vi "Save Image Module.vi"(8 "error in":errorcluster, 10 "Data":u64[](array[numeric]), 11 "Mode":T1) -> (0 "error out":errorcluster, 3 "File Open?":bool)   [LabVIEW 2013]
uses:
  Save Image Module Enum.ctl
  Debug/Debug Settings FG Enum.ctl
  Image Acquisition/Image Acquisition Settings FG Enum.ctl
  Image Processing/Mask ROI FG Enum.ctl
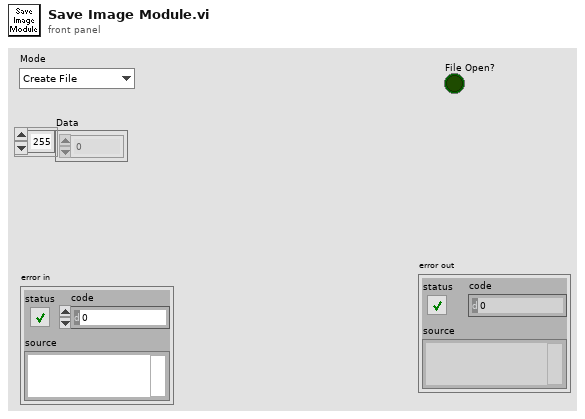
[diagram p1: front panel]
types:
  T1 = typedef "Save Image Module Enum.ctl" = enum16{"Create File", "Write to File", "Status", "Close File"}
  T2 = typedef "Debug Settings FG Enum.ctl" = enum16{"Read", "Write"}
  T3 = typedef "Debug Settings Cluster.ctl" = cluster{"Save Images?":bool, "Save Image Path":path}
  T4 = typedef "Mask ROI FG Enum.ctl" = enum16{"Read", "Write", "Enable Background", "Disable Background"}
  T5 = typedef "Image Acquisition Settings FG Enum.ctl" = enum16{"Read", "Write"}
  T6 = enum16{"open", "replace", "create", "open or create", "replace or create", "replace or create with confirmation"}
  T7 = typedef "Acquisition Settings Cluster.ctl" = cluster{"Image Width":u32, "Image Height":u32, "Frames To Acquire":u32, "Signal Mapping":enum8{"Standard", "Basler 10-tap", "Vosskühler 10-tap"}, "DMA Buffer Size\n(In Images)":u32}
  T8 = typedef "Mask ROI Cluster.ctl" = cluster{"left annulus":T9, "right annulus":T9, "Threshold Range":cluster{"Lower value":dbl, "Upper value":dbl}, "[Avg BG]":u8[], "Number of Sectors":u8, "Left ROI":T10, "Right ROI":T10, "Left Start Angle Duty Cycle":fxp<+,8,0>, "Left End Angle Duty Cycle":fxp<+,8,0>, "Right End Angle Duty Cycle":fxp<+,8,0>, "Right Start Angle Duty Cycle":fxp<+,8,0>, "[Sector ROIs]":T10[], "Consecutive Sector Threshold":u8}
  T9 = typedef "IMAQ Circle" = cluster{"Center X":i32, "Center Y":i32, "Inner Radius":i32, "Outer Radius":i32, "Start Angle":dbl, "End Angle":dbl}
  T10 = typedef "ROI Descriptor" = cluster{"Global Rectangle":i32[], "Contours":cluster{"ID":enum32{"External", "Internal"}, "Type":u32, "Coordinates":i32[]}[]}
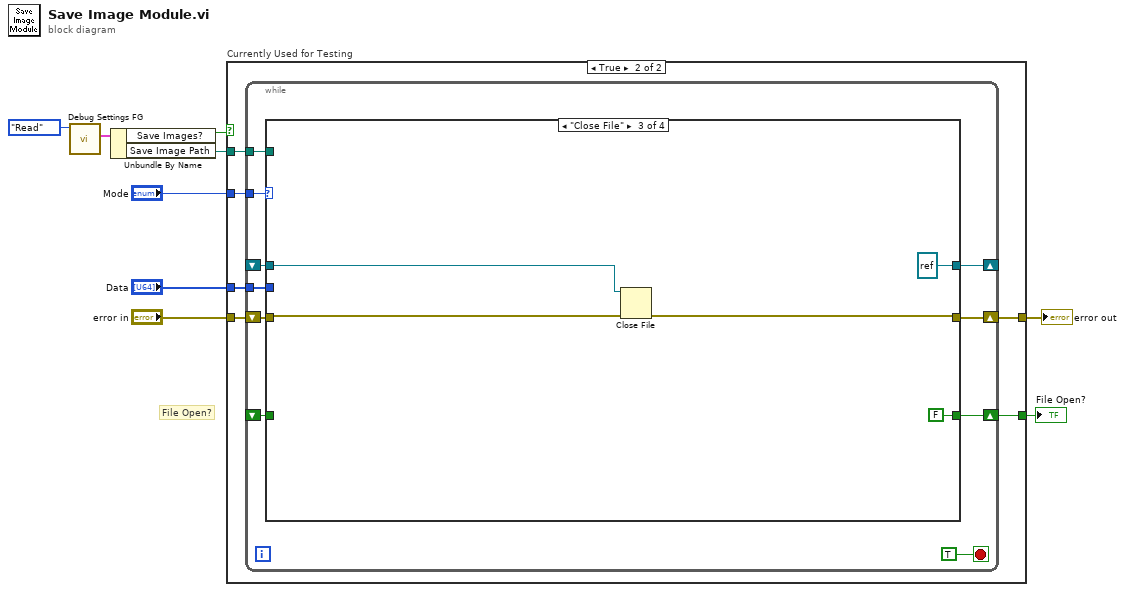
[diagram p0: block diagram]
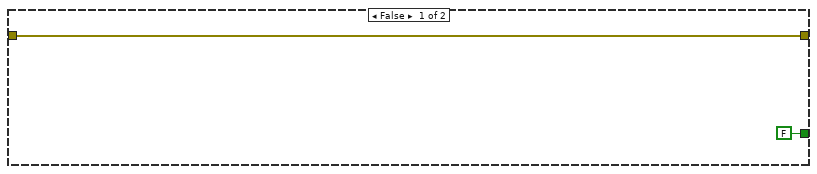
[diagram p2: hidden frame]
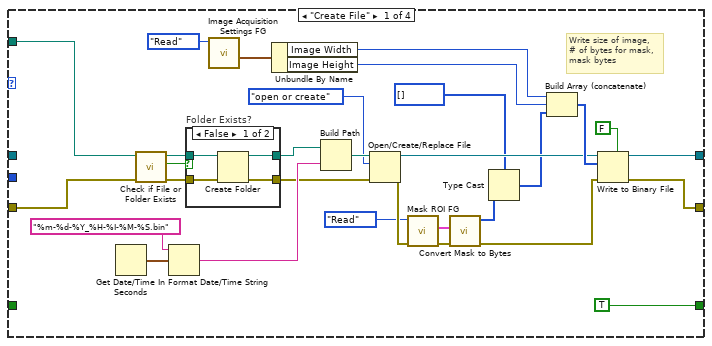
[diagram p3: hidden frame]
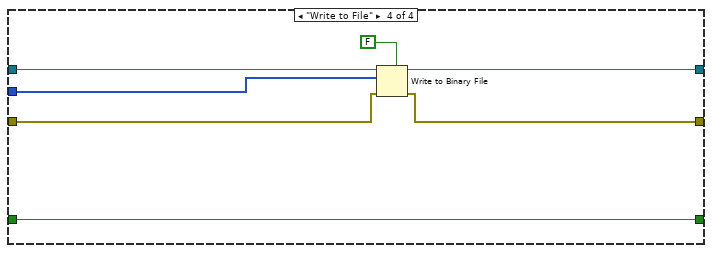
[diagram p6: hidden frame]
diagram:
  # "File Open?"
  n1 = call "Debug Settings FG.vi"("Operation"=Debug_Settings_FG_Enum."Read") -> ("Debug Settings Out"=w5:T3)  [unwired: 9 in, 1 out]
  n2 = Unbundle By Name(w5) -> ("Save Images?"=w4:bool, "Save Image Path"=w2:path)
  n3 = case "Currently Used for Testing" shown="True" w4 {
    tunnel: "Mode" -> [_ w17]
    tunnel: "error in" -> [w11 w16]
    tunnel: [w11 w15] -> w7
    tunnel: "Data" -> [_ w14]
    tunnel: w2 -> [_ w13]
    tunnel: [FALSE w12] -> w1
    frame False {
    }
    frame True {
      n4 = while {
        tunnel: w17 -> [w26]
        shift-right: [w23] -> w15
        shift-left: w16 -> [w25]
        shift-right: [w24] -> _
        shift-left: _ -> [w22]
        tunnel: w14 -> [w21]
        tunnel: w13 -> [w20]
        shift-right: [w19] -> w12
        shift-left: _ -> [w18]
        stop <- TRUE stop-if-true
        n5 = case shown="\"Close File\"" w26 {
          tunnel: w25 -> [w38 w65 w71 w77]
          tunnel: [w41 w66 refnum<file> refnum ("refnum out") w75] -> w24
          tunnel: [w40 w65 w70 w76] -> w23
          tunnel: w22 -> [_ w66 w69 w78]
          tunnel: w21 -> [_ _ _ w73]
          tunnel: w20 -> [w39 _ _ _]
          tunnel: [TRUE w64 FALSE w72] -> w19
          tunnel: w18 -> [_ w64 _ w72]
          frame "Create File" {
            # "Write size of image,\n# of bytes for mask,\nmask bytes"
            n6 = Get Date/Time In Seconds() -> (seconds since 1Jan1904=w55:timestamp)
            n7 = call <vilib>:"Check if File or Folder Exists.vi"("error in (no error)"=w38, "path"=w39) -> ("error out"=w52:errorcluster, "file or folder exists?"=w54:bool, "dup path"=w53:path)  [unwired: 7 in]
            n8 = Format Date/Time String(time format string (%c)="%m-%d-%Y_%H-%I-%M-%S.bin", seconds (now)=w55) -> (date/time string=w57:string)  [unwired: 1 in]
            n9 = case "Folder Exists?" shown="False" w54 {
              tunnel: w53 -> [w61 w63]
              tunnel: w52 -> [w60 w62]
              tunnel: [w59 w62] -> w48
              tunnel: [w58 w63] -> w51
              frame False {
                n10 = Create Folder(path (use dialog)=w61, error in=w60) -> (created path=w58:path, error out=w59:errorcluster)  [unwired: 1 in, 1 out]
              }
              frame True {
              }
            }
            n11 = call "Image Acquisition Settings FG.vi"("Operation"=Image_Acquisition_Settings_FG_Enum."Read") -> ("Acquisition Settings Out"=w46:T7)  [unwired: 9 in, 1 out]
            n12 = Unbundle By Name(w46) -> ("Image Width"=w45:u32, "Image Height"=w44:u32)
            n13 = Build Path(base path=w51, name or relative path=w57) -> (appended path=w50:path)
            n14 = Open/Create/Replace File(file path (use dialog)=w50, error in=w48, operation (0:open)=T6."open or create") -> (refnum out=w36:refnum<file>, error out=w37:errorcluster)  [unwired: 3 in, 1 out]
            n15 = call "Mask ROI FG.vi"("error in (no error)"=w37, "Operation"=Mask_ROI_FG_Enum."Read") -> ("error out"=w34:errorcluster, "Mask ROI Out"=w33:T8)  [unwired: 8 in]
            n16 = call "Convert Mask to Bytes.vi"("error in (no error)"=w34, "Mask ROI In"=w33) -> ("error out"=w32:errorcluster, "Mask Bytes Out"=w30:u8[])  [unwired: 7 in, 1 out]
            n17 = Type Cast(type=u32[] [], x=w30) -> (*(type *) &x=w29:u32[])
            n18 = Build Array (concatenate)(w45, w44, w29) -> (w42:u32[])
            n19 = Write to Binary File(file (use dialog)=w36, data=w42, error in=w32, 5:FALSE ("prepend array or string size? (T)")) -> (refnum out=w41:refnum<file>, error out=w40:errorcluster)  [unwired: 2 in, 1 out]
          }
          frame "Status" {
          }
          frame "Close File" {
            n20 = Close File(refnum=w69, error in=w71) -> (error out=w70:errorcluster)  [unwired: 1 out]
          }
          frame "Write to File" {
            n21 = Write to Binary File(file (use dialog)=w78, data=w73, error in=w77, 5:FALSE ("prepend array or string size? (T)")) -> (refnum out=w75:refnum<file>, error out=w76:errorcluster)  [unwired: 2 in, 1 out]
          }
        }
      }
    }
  }
  "error out" <- w7
  "File Open?" <- w1
